vi "Reduce Files.vi"() -> ()   [LabVIEW 2015]
uses:
  <userlib>/_OpenG.lib/file/file.llb/Strip Path Extension - String__ogtk.vi
panel:
  out "spreadsheet string":string
  in  "Delete?":bool
  out "array 3":string[](array[string])
  out "array 2":string[](array[string])
  out "array":string[](array[string])
  # "UFileCrc32"
  # "INPUT: at blockdiagramm"
  # "Look out: some  *.pas files  do  not have a *.dcu file\nwhen included like\n{$I I_Connector_Diff.pas}"
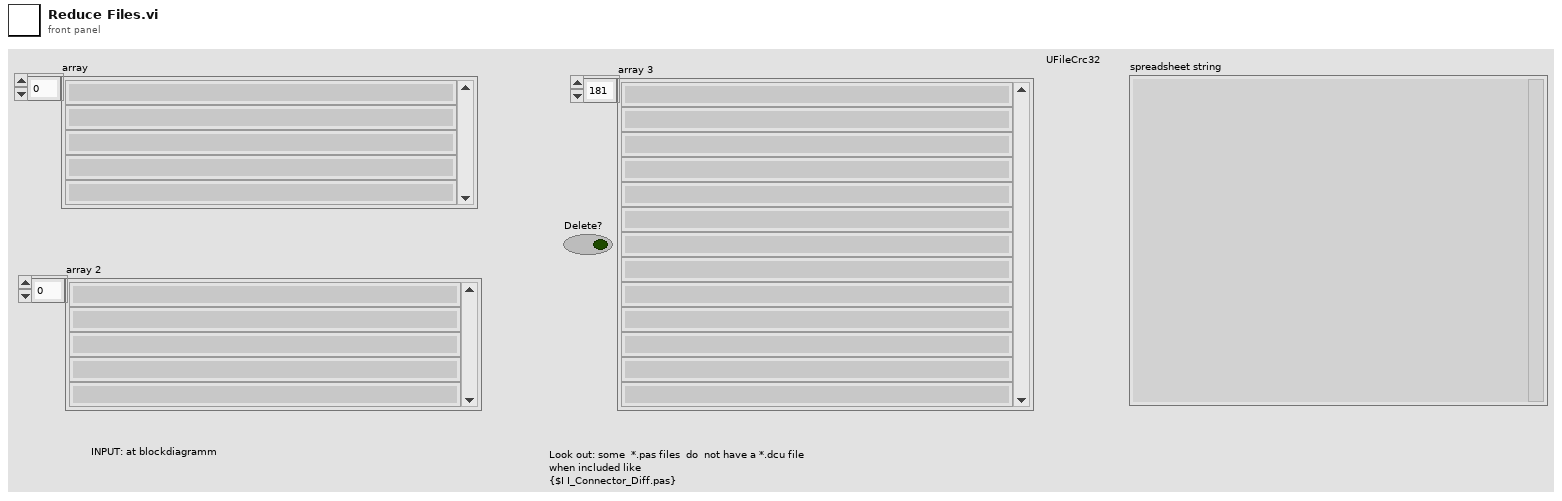
[diagram p1: front panel]
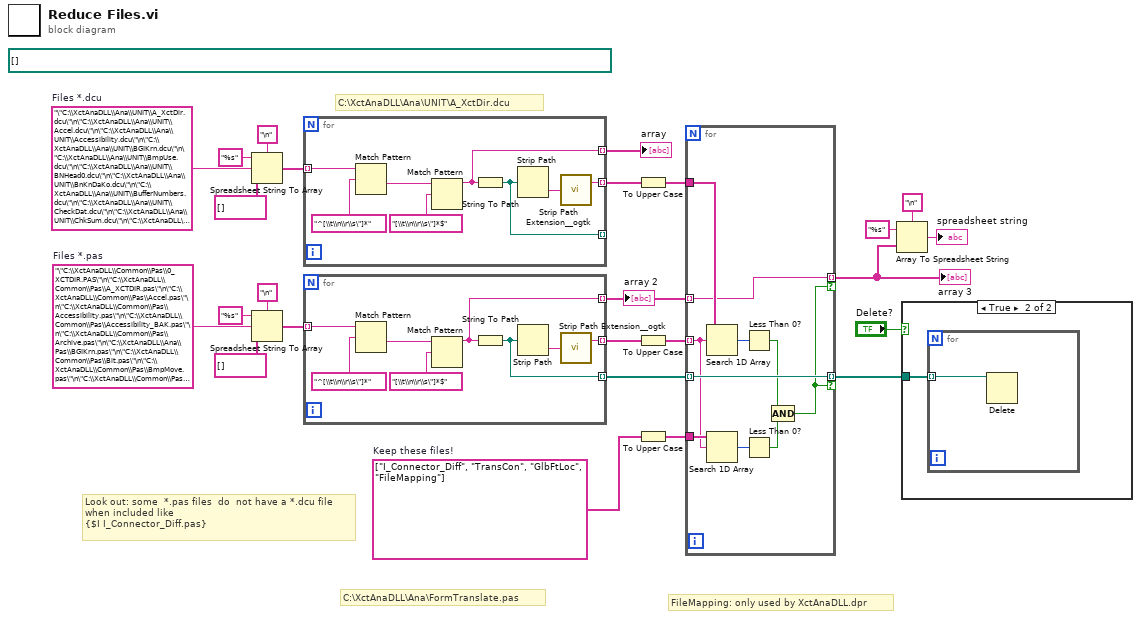
[diagram p0: block diagram]
diagram:
  w2 = string[] ["I_Connector_Diff", "TransCon", "GlbFtLoc", "FileMapping"]  # Keep these files!
  w19 = "\"C:\\XctAnaDLL\\Ana\\UNIT\\A_XctDir.dcu\"\n\"C:\\XctAnaDLL\\Ana\\UNIT\\Accel.dcu\"\n\"C:\\XctAnaDLL\\Ana\\UNIT\\Accessibility.dcu\"\n\"C:\\XctAnaDLL\\Ana\\UNIT\\BGIKrn.dcu\"\n\"C:\\XctAnaDLL\\Ana\\UNIT\\BmpUse.dcu\"\n\"C:\\XctAnaDLL\\Ana\\UNIT\\BNHead0.dcu\"\n\"C:\\XctAnaDLL\\Ana\\UNIT\\BnKnDaKo.dcu\"\n\"C:\\XctAnaDLL\\Ana\\UNIT\\BufferNumbers.dcu\"\n\"C:\\XctAnaDLL\\Ana\\UNIT\\CheckDat.dcu\"\n\"C:\\XctAnaDLL\\Ana\\UNIT\\ChkSum.dcu\"\n\"C:\\XctAnaDLL\\Ana\\UNIT\\ClientViewXctImagesUnit.dcu\"\n\"C:\\XctAnaDLL\\Ana\\UNIT\\ClipBrdUse.dcu\"\n\"C:\\XctAnaDLL\\Ana\\UNIT\\CodeFind.dcu\"\n\"C:\\XctAnaDLL\\Ana\\UNIT\\ColorDlgUse.dcu\"\n\"C:\\XctAnaDLL\\Ana\\UNIT\\ColorModels.dcu\"\n\"C:\\XctAnaDLL\\Ana\\UNIT\\ColorsPlus.dcu\"\n\"C:\\XctAnaDLL\\Ana\\UNIT\\ComNames.dcu\"\n\"C:\\XctAnaDLL\\Ana\\UNIT\\CRT.dcu\"\n\"C:\\XctAnaDLL\\Ana\\UNIT\\DebugForm.dcu\"\n\"C:\\XctAnaDLL\\Ana\\UNIT\\DefHTMLOpts.dcu\"\n\"C:\\XctAnaDLL\\Ana\\UNIT\\DelphiCrt.dcu\"\n\"C:\\XctAnaDLL\\Ana\\UNIT\\DialogsSecure.dcu\"\n\"C:\\XctAnaDLL\\Ana\\UNIT\\DIBTools.dcu\"\n\"C:\\XctAnaDLL\\Ana\\UNIT\\Dos.dcu\"\n\"C:\\XctAnaDLL\\Ana\\UNIT\\DosTimer.dcu\"\n\"C:\\XctAnaDLL\\Ana\\UNIT\\Draw.dcu\"\n\"C:\\XctAnaDLL\\Ana\\UNIT\\EE_Param.dcu\"\n\"C:\\XctAnaDLL\\Ana\\UNIT\\ErrConst.dcu\"\n\"C:\\XctAnaDLL\\Ana\\UNIT\\EventLogs.dcu\"\n\"C:\\XctAnaDLL\\Ana\\UNIT\\ExitTool.dcu\"\n\"C:\\XctAnaDLL\\Ana\\UNIT\\FemGlb.dcu\"\n\"C:\\XctAnaDLL\\Ana\\UNIT\\FemurPcForm1.dcu\"\n\"C:\\XctAnaDLL\\Ana\\UNIT\\FileUtils.dcu\"\n\"C:\\XctAnaDLL\\Ana\\UNIT\\FindEdge.dcu\"\n\"C:\\XctAnaDLL\\Ana\\UNIT\\FormatedList.dcu\"\n\"C:\\XctAnaDLL\\Ana\\UNIT\\FramePaint.dcu\"\n\"C:\\XctAnaDLL\\Ana\\UNIT\\frmBnLockPassWd.dcu\"\n\"C:\\XctAnaDLL\\Ana\\UNIT\\FrmXCTAbout.dcu\"\n\"C:\\XctAnaDLL\\Ana\\UNIT\\GlbDecs.dcu\"\n\"C:\\XctAnaDLL\\Ana\\UNIT\\GlbFT.dcu\"\n\"C:\\XctAnaDLL\\Ana\\UNIT\\GlbPath.dcu\"\n\"C:\\XctAnaDLL\\Ana\\UNIT\\GlbTools.dcu\"\n\"C:\\XctAnaDLL\\Ana\\UNIT\\GlbType.dcu\"\n\"C:\\XctAnaDLL\\Ana\\UNIT\\Graph0.dcu\"\n\"C:\\XctAnaDLL\\Ana\\UNIT\\GraphGlb.dcu\"\n\"C:\\XctAnaDLL\\Ana\\UNIT\\GraphicsExt.dcu\"\n\"C:\\XctAnaDLL\\Ana\\UNIT\\IOTools.dcu\"\n\"C:\\XctAnaDLL\\Ana\\UNIT\\JpgUse.dcu\"\n\"C:\\XctAnaDLL\\Ana\\UNIT\\KeyCodes.dcu\"\n\"C:\\XctAnaDLL\\Ana\\UNIT\\KeyState.dcu\"\n\"C:\\XctAnaDLL\\Ana\\UNIT\\Kn_Debug.dcu\"\n\"C:\\XctAnaDLL\\Ana\\UNIT\\KN_Err.dcu\"\n\"C:\\XctAnaDLL\\Ana\\UNIT\\KN_HLP.dcu\"\n\"C:\\XctAnaDLL\\Ana\\UNIT\\KN_Math.dcu\"\n\"C:\\XctAnaDLL\\Ana\\UNIT\\KN_MI.dcu\"\n\"C:\\XctAnaDLL\\Ana\\UNIT\\KN_NCONT.dcu\"\n\"C:\\XctAnaDLL\\Ana\\UNIT\\Kn_NGlb.dcu\"\n\"C:\\XctAnaDLL\\Ana\\UNIT\\KN_NSPLI.dcu\"\n\"C:\\XctAnaDLL\\Ana\\UNIT\\KN_PRINT.dcu\"\n\"C:\\XctAnaDLL\\Ana\\UNIT\\KN_ROI.dcu\"\n\"C:\\XctAnaDLL\\Ana\\UNIT\\KN_SetUp.dcu\"\n\"C:\\XctAnaDLL\\Ana\\UNIT\\KN_Slc.dcu\"\n\"C:\\XctAnaDLL\\Ana\\UNIT\\KN_TOPAZ.dcu\"\n\"C:\\XctAnaDLL\\Ana\\UNIT\\KnMulti.dcu\"\n\"C:\\XctAnaDLL\\Ana\\UNIT\\LabViewAna.dcu\"\n\"C:\\XctAnaDLL\\Ana\\UNIT\\LinTick0.dcu\"\n\"C:\\XctAnaDLL\\Ana\\UNIT\\LPCF_GLB.dcu\"\n\"C:\\XctAnaDLL\\Ana\\UNIT\\MemTools.dcu\"\n\"C:\\XctAnaDLL\\Ana\\UNIT\\MenuIds.dcu\"\n\"C:\\XctAnaDLL\\Ana\\UNIT\\MenuProc.dcu\"\n\"C:\\XctAnaDLL\\Ana\\UNIT\\MenuTool.dcu\"\n\"C:\\XctAnaDLL\\Ana\\UNIT\\MsgBox.dcu\"\n\"C:\\XctAnaDLL\\Ana\\UNIT\\Objects.dcu\"\n\"C:\\XctAnaDLL\\Ana\\UNIT\\Objects0.dcu\"\n\"C:\\XctAnaDLL\\Ana\\UNIT\\OrientDirUse.dcu\"\n\"C:\\XctAnaDLL\\Ana\\UNIT\\PCX.dcu\"\n\"C:\\XctAnaDLL\\Ana\\UNIT\\PntMath.dcu\"\n\"C:\\XctAnaDLL\\Ana\\UNIT\\PowerButton.dcu\"\n\"C:\\XctAnaDLL\\Ana\\UNIT\\PrinterGlb.dcu\"\n\"C:\\XctAnaDLL\\Ana\\UNIT\\PrintersFpu.dcu\"\n\"C:\\XctAnaDLL\\Ana\\UNIT\\PrintForm.dcu\"\n\"C:\\XctAnaDLL\\Ana\\UNIT\\ProgressBars.dcu\"\n\"C:\\XctAnaDLL\\Ana\\UNIT\\ReadPar.dcu\"\n\"C:\\XctAnaDLL\\Ana\\UNIT\\RectGlb.dcu\"\n\"C:\\XctAnaDLL\\Ana\\UNIT\\RoiDialog.dcu\"\n\"C:\\XctAnaDLL\\Ana\\UNIT\\RoiDialogTools.dcu\"\n\"C:\\XctAnaDLL\\Ana\\UNIT\\RoiMath.dcu\"\n\"C:\\XctAnaDLL\\Ana\\UNIT\\ScanIo0.dcu\"\n\"C:\\XctAnaDLL\\Ana\\UNIT\\SCRConst.dcu\"\n\"C:\\XctAnaDLL\\Ana\\UNIT\\SelectForm.dcu\"\n\"C:\\XctAnaDLL\\Ana\\UNIT\\SetDecimalPoint.dcu\"\n\"C:\\XctAnaDLL\\Ana\\UNIT\\SpinEdit2.dcu\"\n\"C:\\XctAnaDLL\\Ana\\UNIT\\StrTool.dcu\"\n\"C:\\XctAnaDLL\\Ana\\UNIT\\THaloEdi.dcu\"\n\"C:\\XctAnaDLL\\Ana\\UNIT\\THaloWin.dcu\"\n\"C:\\XctAnaDLL\\Ana\\UNIT\\ThreadView.dcu\"\n\"C:\\XctAnaDLL\\Ana\\UNIT\\TKeyApp.dcu\"\n\"C:\\XctAnaDLL\\Ana\\UNIT\\TMathobj.dcu\"\n\"C:\\XctAnaDLL\\Ana\\UNIT\\TMenuApp.dcu\"\n\"C:\\XctAnaDLL\\Ana\\UNIT\\TNHTOOL.dcu\"\n\"C:\\XctAnaDLL\\Ana\\UNIT\\Tools.dcu\"\n\"C:\\XctAnaDLL\\Ana\\UNIT\\Translate.dcu\"\n\"C:\\XctAnaDLL\\Ana\\UNIT\\TransX.dcu\"\n\"C:\\XctAnaDLL\\Ana\\UNIT\\TurbExt1.dcu\"\n\"C:\\XctAnaDLL\\Ana\\UNIT\\TurboToDelphi.dcu\"\n\"C:\\XctAnaDLL\\Ana\\UNIT\\TypesUse.dcu\"\n\"C:\\XctAnaDLL\\Ana\\UNIT\\UBnLockWin.dcu\"\n\"C:\\XctAnaDLL\\Ana\\UNIT\\UFileCrc32.dcu\"\n\"C:\\XctAnaDLL\\Ana\\UNIT\\UfrmRefReport.dcu\"\n\"C:\\XctAnaDLL\\Ana\\UNIT\\UfrmShowRef.dcu\"\n\"C:\\XctAnaDLL\\Ana\\UNIT\\UMsgDelay.dcu\"\n\"C:\\XctAnaDLL\\Ana\\UNIT\\UniDIB.dcu\"\n\"C:\\XctAnaDLL\\Ana\\UNIT\\UReadSet.dcu\"\n\"C:\\XctAnaDLL\\Ana\\UNIT\\UseDelphi.dcu\"\n\"C:\\XctAnaDLL\\Ana\\UNIT\\UTA_CBD.dcu\"\n\"C:\\XctAnaDLL\\Ana\\UNIT\\UtAna.dcu\"\n\"C:\\XctAnaDLL\\Ana\\UNIT\\UTAna1.dcu\"\n\"C:\\XctAnaDLL\\Ana\\UNIT\\UTAROI.dcu\"\n\"C:\\XctAnaDLL\\Ana\\UNIT\\UTArray.dcu\"\n\"C:\\XctAnaDLL\\Ana\\UNIT\\UTBuffer.dcu\"\n\"C:\\XctAnaDLL\\Ana\\UNIT\\UTColDlg.dcu\"\n\"C:\\XctAnaDLL\\Ana\\UNIT\\UTColor.dcu\"\n\"C:\\XctAnaDLL\\Ana\\UNIT\\UTDBI.dcu\"\n\"C:\\XctAnaDLL\\Ana\\UNIT\\UtFilt0.dcu\"\n\"C:\\XctAnaDLL\\Ana\\UNIT\\UtFilter.dcu\"\n\"C:\\XctAnaDLL\\Ana\\UNIT\\UTGenOb.dcu\"\n\"C:\\XctAnaDLL\\Ana\\UNIT\\UTGENROI.dcu\"\n\"C:\\XctAnaDLL\\Ana\\UNIT\\UTGrpRes.dcu\"\n\"C:\\XctAnaDLL\\Ana\\UNIT\\UtIni.dcu\"\n\"C:\\XctAnaDLL\\Ana\\UNIT\\UTIP.dcu\"\n\"C:\\XctAnaDLL\\Ana\\UNIT\\UTKnApp.dcu\"\n\"C:\\XctAnaDLL\\Ana\\UNIT\\UTKnApp0.dcu\"\n\"C:\\XctAnaDLL\\Ana\\UNIT\\UTKNAPP1.dcu\"\n\"C:\\XctAnaDLL\\Ana\\UNIT\\UTKNAPP2.dcu\"\n\"C:\\XctAnaDLL\\Ana\\UNIT\\UtKnPane.dcu\"\n\"C:\\XctAnaDLL\\Ana\\UNIT\\UTParam.dcu\"\n\"C:\\XctAnaDLL\\Ana\\UNIT\\UTRef.dcu\"\n\"C:\\XctAnaDLL\\Ana\\UNIT\\UTRes.dcu\"\n\"C:\\XctAnaDLL\\Ana\\UNIT\\UTStd.dcu\"\n\"C:\\XctAnaDLL\\Ana\\UNIT\\VidLine.dcu\"\n\"C:\\XctAnaDLL\\Ana\\UNIT\\ViewQLim.dcu\"\n\"C:\\XctAnaDLL\\Ana\\UNIT\\ViewScreens.dcu\"\n\"C:\\XctAnaDLL\\Ana\\UNIT\\ViewXctImages.dcu\"\n\"C:\\XctAnaDLL\\Ana\\UNIT\\ViewXctServerClientGlb.dcu\"\n\"C:\\XctAnaDLL\\Ana\\UNIT\\WindowsEx.dcu\"\n\"C:\\XctAnaDLL\\Ana\\UNIT\\WinTmr.dcu\"\n\"C:\\XctAnaDLL\\Ana\\UNIT\\WinTools.dcu\"\n\"C:\\XctAnaDLL\\Ana\\UNIT\\WM_AddMessages.dcu\"\n\"C:\\XctAnaDLL\\Ana\\UNIT\\XctVersion.dcu\"\n\"C:\\XctAnaDLL\\Ana\\UNIT\\XGlb.dcu\"\n\"C:\\XctAnaDLL\\Ana\\UNIT\\XMeasGrp.dcu\""  # Files *.dcu
  w18 = "\"C:\\XctAnaDLL\\Common\\Pas\\0_XCTDIR.PAS\"\n\"C:\\XctAnaDLL\\Common\\Pas\\A_XCTDIR.pas\"\n\"C:\\XctAnaDLL\\Common\\Pas\\Accel.pas\"\n\"C:\\XctAnaDLL\\Common\\Pas\\Accessibility.pas\"\n\"C:\\XctAnaDLL\\Common\\Pas\\Accessibility_BAK.pas\"\n\"C:\\XctAnaDLL\\Common\\Pas\\Archive.pas\"\n\"C:\\XctAnaDLL\\Ana\\Pas\\BGIKrn.pas\"\n\"C:\\XctAnaDLL\\Common\\Pas\\Bit.pas\"\n\"C:\\XctAnaDLL\\Common\\Pas\\BmpMove.pas\"\n\"C:\\XctAnaDLL\\Common\\Pas\\BmpStack.pas\"\n\"C:\\XctAnaDLL\\Common\\Pas\\BmpUse.pas\"\n\"C:\\XctAnaDLL\\Common\\Pas\\BNHead0.pas\"\n\"C:\\XctAnaDLL\\Ana\\Pas\\BNKEY0.pas\"\n\"C:\\XctAnaDLL\\Ana\\Pas\\BnKnDaKo.pas\"\n\"C:\\XctAnaDLL\\Ana\\Pas\\BNLOCK.pas\"\n\"C:\\XctAnaDLL\\Ana\\Pas\\BufferNumbers.pas\"\n\"C:\\XctAnaDLL\\Ana\\Pas\\BufferNumbers_2.pas\"\n\"C:\\XctAnaDLL\\Ana\\Pas\\Calc.pas\"\n\"C:\\XctAnaDLL\\Common\\Pas\\CheckDat.pas\"\n\"C:\\XctAnaDLL\\Common\\Pas\\CheckPrevious.pas\"\n\"C:\\XctAnaDLL\\Ana\\Pas\\CHK540UP.PAS\"\n\"C:\\XctAnaDLL\\Common\\Pas\\ChkSum.pas\"\n\"C:\\XctAnaDLL\\Ana\\Pas\\ChngSide.pas\"\n\"C:\\XctAnaDLL\\Common\\Pas\\ClientViewXctImagesUnit.pas\"\n\"C:\\XctAnaDLL\\Common\\Pas\\ClipBrdUse.pas\"\n\"C:\\XctAnaDLL\\Ana\\Pas\\cmConst.pas\"\n\"C:\\XctAnaDLL\\Ana\\Pas\\CMDPARAM.PAS\"\n\"C:\\XctAnaDLL\\Common\\Pas\\CodeFind.pas\"\n\"C:\\XctAnaDLL\\Common\\Pas\\ColorDlgUse.pas\"\n\"C:\\XctAnaDLL\\Common\\Pas\\ColorModels.pas\"\n\"C:\\XctAnaDLL\\Common\\Pas\\ColorsPlus.pas\"\n\"C:\\XctAnaDLL\\Info\\TempTest\\COMAC000_Msk.pas\"\n\"C:\\XctAnaDLL\\Info\\TempTest\\COMACFEM_Msk.pas\"\n\"C:\\XctAnaDLL\\Common\\Pas\\ComNames.pas\"\n\"C:\\XctAnaDLL\\Common\\Pas\\ComparePathes.pas\"\n\"C:\\XctAnaDLL\\Common\\Pas\\Complexs.pas\"\n\"C:\\XctAnaDLL\\Ana\\Pas\\CONF.PAS\"\n\"C:\\XctAnaDLL\\Common\\Pas\\ControlsUse.pas\"\n\"C:\\XctAnaDLL\\Common\\Pas\\Crt.pas\"\n\"C:\\XctAnaDLL\\Ana\\Pas\\CSV2PAL.pas\"\n\"C:\\XctAnaDLL\\Ana\\Pas\\csvread.pas\"\n\"C:\\XctAnaDLL\\Ana\\Pas\\CSVSTAT.pas\"\n\"C:\\XctAnaDLL\\Ana\\Pas\\CVDOSTXT.PAS\"\n\"C:\\XctAnaDLL\\Common\\Pas\\DataBaseXct.pas\"\n\"C:\\XctAnaDLL\\Common\\Pas\\DebInit.pas\"\n\"C:\\XctAnaDLL\\Common\\Pas\\DebugForm.pas\"\n\"C:\\XctAnaDLL\\Ana\\Pas\\DefDrvs.pas\"\n\"C:\\XctAnaDLL\\Common\\Pas\\DefHTMLOpts.pas\"\n\"C:\\XctAnaDLL\\Common\\Pas\\DelphiCrt.pas\"\n\"C:\\XctAnaDLL\\Common\\Pas\\DialogsSecure.pas\"\n\"C:\\XctAnaDLL\\Common\\Pas\\DIBTools.pas\"\n\"C:\\XctAnaDLL\\Common\\Pas\\DirTool.pas\"\n\"C:\\XctAnaDLL\\Common\\Pas\\DiskTyp.pas\"\n\"C:\\XctAnaDLL\\Common\\Pas\\DlgDeltaTime.pas\"\n\"C:\\XctAnaDLL\\Ana\\Pas\\Do540up.pas\"\n\"C:\\XctAnaDLL\\Ana\\Pas\\DoModify.pas\"\n\"C:\\XctAnaDLL\\Common\\Pas\\Dos.pas\"\n\"C:\\XctAnaDLL\\Common\\Pas\\DosGlb.pas\"\n\"C:\\XctAnaDLL\\Common\\Pas\\DosTimer.pas\"\n\"C:\\XctAnaDLL\\Common\\Pas\\Draw.pas\"\n\"C:\\XctAnaDLL\\Common\\Pas\\DrawGridDialog.pas\"\n\"C:\\XctAnaDLL\\Ana\\Pas\\DUMMY.PAS\"\n\"C:\\XctAnaDLL\\Common\\Pas\\EE_Param.pas\"\n\"C:\\XctAnaDLL\\Common\\Pas\\EE_Param_RW.pas\"\n\"C:\\XctAnaDLL\\Common\\Pas\\EE_Param_Tools.pas\"\n\"C:\\XctAnaDLL\\Common\\Pas\\ErrConst.pas\"\n\"C:\\XctAnaDLL\\Common\\Pas\\EventLog.pas\"\n\"C:\\XctAnaDLL\\Common\\Pas\\EventLogs.pas\"\n\"C:\\XctAnaDLL\\Ana\\Pas\\ExGraph.pas\"\n\"C:\\XctAnaDLL\\Common\\Pas\\ExitTool.pas\"\n\"C:\\XctAnaDLL\\Ana\\Pas\\EXTPLUS.pas\"\n\"C:\\XctAnaDLL\\Ana\\Pas\\FCOUNT.pas\"\n\"C:\\XctAnaDLL\\Common\\Pas\\FemGlb.pas\"\n\"C:\\XctAnaDLL\\Common\\Pas\\FemurPcForm1.pas\"\n\"C:\\XctAnaDLL\\Common\\Pas\\FFTs.pas\"\n\"C:\\XctAnaDLL\\Delphi\\FileMapping.pas\"\n\"C:\\XctAnaDLL\\Common\\Pas\\FileUtils.pas\"\n\"C:\\XctAnaDLL\\Ana\\Pas\\FindEdge.pas\"\n\"C:\\XctAnaDLL\\Common\\Pas\\FirFilter.pas\"\n\"C:\\XctAnaDLL\\Common\\Pas\\FormatedList.pas\"\n\"C:\\XctAnaDLL\\Common\\Pas\\FormatTools.pas\"\n\"C:\\XctAnaDLL\\Ana\\Pas\\formLoopEdit.pas\"\n\"C:\\XctAnaDLL\\Common\\Pas\\FormMountImage.pas\"\n\"C:\\XctAnaDLL\\Ana\\FormTranslate.pas\"\n\"C:\\XctAnaDLL\\Common\\Pas\\Fourier.pas\"\n\"C:\\XctAnaDLL\\Common\\Pas\\FramePaint.pas\"\n\"C:\\XctAnaDLL\\Common\\Pas\\Frames.pas\"\n\"C:\\XctAnaDLL\\Common\\Pas\\FrameScrolledImage.pas\"\n\"C:\\XctAnaDLL\\Common\\Pas\\FrameScrolledImageTool.pas\"\n\"C:\\XctAnaDLL\\Common\\Pas\\FrameToolRect.pas\"\n\"C:\\XctAnaDLL\\Common\\Pas\\frmBnLockPassWd.pas\"\n\"C:\\XctAnaDLL\\Common\\Pas\\frmHexEdit_U.pas\"\n\"C:\\XctAnaDLL\\Common\\Pas\\frmImage.pas\"\n\"C:\\XctAnaDLL\\Common\\Pas\\frmOptsFilesHyperlink.pas\"\n\"C:\\XctAnaDLL\\Common\\Pas\\FrmXCTAbout.pas\"\n\"C:\\XctAnaDLL\\Common\\Pas\\GdiPlusUse.pas\"\n\"C:\\XctAnaDLL\\Common\\Pas\\GeoTools.pas\"\n\"C:\\XctAnaDLL\\Common\\Pas\\GetMovit.pas\"\n\"C:\\XctAnaDLL\\Common\\Pas\\GetTast.pas\"\n\"C:\\XctAnaDLL\\Common\\Pas\\GIFImage.pas\"\n\"C:\\XctAnaDLL\\Common\\Pas\\Glb.pas\"\n\"C:\\XctAnaDLL\\Common\\Pas\\GlbDecs.pas\"\n\"C:\\XctAnaDLL\\Common\\Pas\\GlbFT.pas\"\n\"C:\\XctAnaDLL\\Ana\\Pas\\GlbFtLoc.Pas\"\n\"C:\\XctAnaDLL\\Common\\Pas\\GlbFtLoc.Pas\"\n\"C:\\XctAnaDLL\\Common\\Pas\\GlbHotKey.pas\"\n\"C:\\XctAnaDLL\\Common\\Pas\\GlbKey.pas\"\n\"C:\\XctAnaDLL\\Common\\Pas\\GlbPath.pas\"\n\"C:\\XctAnaDLL\\Common\\Pas\\Glbtools.pas\"\n\"C:\\XctAnaDLL\\Common\\Pas\\GlbType.pas\"\n\"C:\\XctAnaDLL\\Ana\\Pas\\GoXctDir.pas\"\n\"C:\\XctAnaDLL\\Common\\Pas\\Gr_Crt.pas\"\n\"C:\\XctAnaDLL\\Common\\Pas\\Graph0.pas\"\n\"C:\\XctAnaDLL\\Common\\Pas\\GraphGlb.pas\"\n\"C:\\XctAnaDLL\\Common\\Pas\\GraphicsExt.pas\"\n\"C:\\XctAnaDLL\\Common\\Pas\\GridBasic.pas\"\n\"C:\\XctAnaDLL\\Ana\\Pas\\HelpFile.pas\"\n\"C:\\XctAnaDLL\\Common\\Pas\\I_Connector_Diff.pas\"\n\"C:\\XctAnaDLL\\Common\\Pas\\IfTool.pas\"\n\"C:\\XctAnaDLL\\Common\\Pas\\ImgBuf.pas\"\n\"C:\\XctAnaDLL\\Common\\Pas\\ImgMeasTools.pas\"\n\"C:\\XctAnaDLL\\Common\\Pas\\ImgOverview.pas\"\n\"C:\\XctAnaDLL\\Common\\Pas\\IniFilesUse.pas\"\n\"C:\\XctAnaDLL\\Common\\Pas\\IntChar.pas\"\n\"C:\\XctAnaDLL\\Ana\\Pas\\Intopaz.pas\"\n\"C:\\XctAnaDLL\\Common\\Pas\\IoErr.pas\"\n\"C:\\XctAnaDLL\\Common\\Pas\\IOTools.pas\"\n\"C:\\XctAnaDLL\\Common\\Pas\\JobParameter.pas\"\n\"C:\\XctAnaDLL\\JPEG\\jpeg.pas\"\n\"C:\\XctAnaDLL\\Common\\Pas\\JpgUse.pas\"\n\"C:\\XctAnaDLL\\Common\\Pas\\KeyCodes.pas\"\n\"C:\\XctAnaDLL\\Ana\\Pas\\Keys.pas\"\n\"C:\\XctAnaDLL\\Common\\Pas\\KeyState.pas\"\n\"C:\\XctAnaDLL\\Ana\\Pas\\Kn_Debug.pas\"\n\"C:\\XctAnaDLL\\Ana\\Pas\\KN_Err.pas\"\n\"C:\\XctAnaDLL\\Ana\\Pas\\KN_HLP.pas\"\n\"C:\\XctAnaDLL\\Ana\\Pas\\KN_Intpz.pas\"\n\"C:\\XctAnaDLL\\Ana\\Pas\\Kn_Math.pas\"\n\"C:\\XctAnaDLL\\Ana\\Pas\\KN_MI.pas\"\n\"C:\\XctAnaDLL\\Ana\\Pas\\KN_NCONT.pas\"\n\"C:\\XctAnaDLL\\Ana\\Pas\\Kn_NGlb.pas\"\n\"C:\\XctAnaDLL\\Ana\\Pas\\KN_NSPLI.pas\"\n\"C:\\XctAnaDLL\\Ana\\Pas\\KN_PRINT.pas\"\n\"C:\\XctAnaDLL\\Ana\\Pas\\KN_ROI.pas\"\n\"C:\\XctAnaDLL\\Ana\\Pas\\KN_SetUp.pas\"\n\"C:\\XctAnaDLL\\Ana\\Pas\\Kn_Slc.pas\"\n\"C:\\XctAnaDLL\\Ana\\Pas\\KN_SLC0.pas\"\n\"C:\\XctAnaDLL\\Ana\\Pas\\KN_TOPAZ.pas\"\n\"C:\\XctAnaDLL\\Ana\\Pas\\KNHLP.pas\"\n\"C:\\XctAnaDLL\\Ana\\Pas\\KnMulti.PAS\"\n\"C:\\XctAnaDLL\\Ana\\Pas\\LabViewAna.pas\"\n\"C:\\XctAnaDLL\\Common\\Pas\\License.pas\"\n\"C:\\XctAnaDLL\\Ana\\Pas\\LicensNo.pas\"\n\"C:\\XctAnaDLL\\Ana\\Pas\\LinTick0.pas\"\n\"C:\\XctAnaDLL\\Ana\\Pas\\loopcfg.pas\"\n\"C:\\XctAnaDLL\\Ana\\Pas\\LoopEditIo.pas\"\n\"C:\\XctAnaDLL\\Ana\\Pas\\LPCF_GLB.pas\"\n\"C:\\XctAnaDLL\\Ana\\Pas\\Lpcftool.pas\"\n\"C:\\XctAnaDLL\\Common\\Pas\\Lv_Tools.pas\"\n\"C:\\XctAnaDLL\\Common\\Pas\\Mail.pas\"\n\"C:\\XctAnaDLL\\Common\\Pas\\MathTool.pas\"\n\"C:\\XctAnaDLL\\Common\\Pas\\MathUse.pas\"\n\"C:\\XctAnaDLL\\Ana\\Pas\\MemTools.pas\"\n\"C:\\XctAnaDLL\\Ana\\Pas\\MenuCons.pas\"\n\"C:\\XctAnaDLL\\Common\\Pas\\MenuIds.pas\"\n\"C:\\XctAnaDLL\\Ana\\Pas\\MenuProc.pas\"\n\"C:\\XctAnaDLL\\Ana\\Pas\\MenuTool.pas\"\n\"C:\\XctAnaDLL\\Common\\Pas\\Minimize.pas\"\n\"C:\\XctAnaDLL\\Common\\Pas\\MsgBox.pas\"\n\"C:\\XctAnaDLL\\Ana\\Pas\\MYREN.pas\"\n\"C:\\XctAnaDLL\\Ana\\Pas\\MyValid.pas\"\n\"C:\\XctAnaDLL\\Ana\\Pas\\NETDEBUG.PAS\"\n\"C:\\XctAnaDLL\\Common\\Pas\\NoXctDir.pas\"\n\"C:\\XctAnaDLL\\Common\\Pas\\Objects.pas\"\n\"C:\\XctAnaDLL\\Common\\Pas\\Objects0.pas\"\n\"C:\\XctAnaDLL\\Common\\Pas\\ObjectsP.pas\"\n\"C:\\XctAnaDLL\\Ana\\Pas\\OEMANSI.PAS\"\n\"C:\\XctAnaDLL\\Ana\\Pas\\OLDVER.pas\"\n\"C:\\XctAnaDLL\\Common\\Pas\\OrientDirUse.pas\"\n\"C:\\XctAnaDLL\\Ana\\Pas\\OVERTYP.pas\"\n\"C:\\XctAnaDLL\\Ana\\Pas\\PAL2CSV.pas\"\n\"C:\\XctAnaDLL\\Common\\Pas\\PauseMsg.pas\"\n\"C:\\XctAnaDLL\\Common\\Pas\\PCX.pas\"\n\"C:\\XctAnaDLL\\Ana\\Pas\\Phan_DLG.pas\"\n\"C:\\XctAnaDLL\\Ana\\Pas\\PifTools.pas\"\n\"C:\\XctAnaDLL\\Common\\Pas\\PntMath.pas\"\n\"C:\\XctAnaDLL\\Common\\Pas\\PowerButton.pas\"\n\"C:\\XctAnaDLL\\Common\\Pas\\PowerButton2.pas\"\n\"C:\\XctAnaDLL\\Common\\Pas\\PrinterGlb.pas\"\n\"C:\\XctAnaDLL\\Common\\Pas\\PrintersFpu.pas\"\n\"C:\\XctAnaDLL\\Common\\Pas\\PrintForm.pas\"\n\"C:\\XctAnaDLL\\Common\\Pas\\PrintFormatted.pas\"\n\"C:\\XctAnaDLL\\Common\\Pas\\PrintTable.pas\"\n\"C:\\XctAnaDLL\\Common\\Pas\\PrnFormatedPages.pas\"\n\"C:\\XctAnaDLL\\Common\\Pas\\ProgressBars.pas\"\n\"C:\\XctAnaDLL\\Common\\Pas\\ReadPar.pas\"\n\"C:\\XctAnaDLL\\Common\\Pas\\Rectangles.pas\"\n\"C:\\XctAnaDLL\\Common\\Pas\\RectGlb.pas\"\n\"C:\\XctAnaDLL\\Ana\\Pas\\Resloop.pas\"\n\"C:\\XctAnaDLL\\Common\\Pas\\ResUse.pas\"\n\"C:\\XctAnaDLL\\Ana\\Pas\\rfdbio.pas\"\n\"C:\\XctAnaDLL\\Common\\Pas\\RichEditUse.pas\"\n\"C:\\XctAnaDLL\\Ana\\Pas\\RoiDialog.pas\"\n\"C:\\XctAnaDLL\\Ana\\Pas\\RoiDialogTools.pas\"\n\"C:\\XctAnaDLL\\Ana\\Pas\\RoiMath.pas\"\n\"C:\\XctAnaDLL\\Common\\Pas\\RollImage.pas\"\n\"C:\\XctAnaDLL\\Common\\Pas\\Round1.pas\"\n\"C:\\XctAnaDLL\\Common\\Pas\\SaverDelphi.pas\"\n\"C:\\XctAnaDLL\\Common\\Pas\\ScanIo0.pas\"\n\"C:\\XctAnaDLL\\Ana\\Pas\\ScrConst.pas\"\n\"C:\\XctAnaDLL\\Ana\\Pas\\Search.pas\"\n\"C:\\XctAnaDLL\\Common\\Pas\\SelectForm.pas\"\n\"C:\\XctAnaDLL\\Common\\Pas\\SerialPortThread.pas\"\n\"C:\\XctAnaDLL\\Common\\Pas\\SerialPortXct.pas\"\n\"C:\\XctAnaDLL\\Common\\Pas\\ServerViewXctImagesUnit.pas\"\n\"C:\\XctAnaDLL\\Ana\\Pas\\SetAvDrv.pas\"\n\"C:\\XctAnaDLL\\Common\\Pas\\SetDecimalPoint.pas\"\n\"C:\\XctAnaDLL\\Ana\\Pas\\SETINI.pas\"\n\"C:\\XctAnaDLL\\Common\\Pas\\ShellLink.pas\"\n\"C:\\XctAnaDLL\\Ana\\Pas\\sparcnst.pas\"\n\"C:\\XctAnaDLL\\Common\\Pas\\SpinEditFloat.pas\"\n\"C:\\XctAnaDLL\\Common\\Pas\\Splines.pas\"\n\"C:\\XctAnaDLL\\Common\\Pas\\StartMeasDialogs.pas\"\n\"C:\\XctAnaDLL\\Common\\Pas\\StreamUse.pas\"\n\"C:\\XctAnaDLL\\Common\\Pas\\StrTool.pas\"\n\"C:\\XctAnaDLL\\Common\\Pas\\SysUse.pas\"\n\"C:\\XctAnaDLL\\Ana\\Pas\\T.PAS\"\n\"C:\\XctAnaDLL\\Ana\\Pas\\T2.PAS\"\n\"C:\\XctAnaDLL\\Ana\\Pas\\T3.PAS\"\n\"C:\\XctAnaDLL\\Ana\\Pas\\T22.PAS\"\n\"C:\\XctAnaDLL\\Ana\\Pas\\TAPP.PAS\"\n\"C:\\XctAnaDLL\\Ana\\Pas\\TAPP2.PAS\"\n\"C:\\XctAnaDLL\\Ana\\Pas\\TDrives.pas\"\n\"C:\\XctAnaDLL\\Common\\Pas\\TeeUse.pas\"\n\"C:\\XctAnaDLL\\Ana\\Pas\\TF.PAS\"\n\"C:\\XctAnaDLL\\Ana\\Pas\\THaloEdi.pas\"\n\"C:\\XctAnaDLL\\Ana\\Pas\\THaloWin.pas\"\n\"C:\\XctAnaDLL\\Common\\Pas\\ThreadView.pas\"\n\"C:\\XctAnaDLL\\Common\\Pas\\TKeyApp.pas\"\n\"C:\\XctAnaDLL\\Ana\\Pas\\TLIST.PAS\"\n\"C:\\XctAnaDLL\\Ana\\Pas\\TMathobj.pas\"\n\"C:\\XctAnaDLL\\Ana\\Pas\\TMenuApp.pas\"\n\"C:\\XctAnaDLL\\Ana\\Pas\\TNHTool.pas\"\n\"C:\\XctAnaDLL\\Common\\Pas\\Tools.pas\"\n\"C:\\XctAnaDLL\\Ana\\Pas\\TRANSCON.PAS\"\n\"C:\\XctAnaDLL\\Common\\Pas\\TRANSCON.PAS\"\n\"C:\\XctAnaDLL\\Common\\Pas\\Translate.pas\"\n\"C:\\XctAnaDLL\\Ana\\TranslateData.pas\"\n\"C:\\XctAnaDLL\\Common\\Pas\\TransX.pas\"\n\"C:\\XctAnaDLL\\Common\\Pas\\TstShlObj.pas\"\n\"C:\\XctAnaDLL\\Ana\\Pas\\TT.PAS\"\n\"C:\\XctAnaDLL\\Ana\\Pas\\TTGRAPHS.PAS\"\n\"C:\\XctAnaDLL\\Ana\\Pas\\TTT.PAS\"\n\"C:\\XctAnaDLL\\Common\\Pas\\TurbExt1.pas\"\n\"C:\\XctAnaDLL\\Common\\Pas\\TurboToDelphi.pas\"\n\"C:\\XctAnaDLL\\Ana\\Pas\\tvedit.pas\"\n\"C:\\XctAnaDLL\\Common\\Pas\\Type_s.pas\"\n\"C:\\XctAnaDLL\\Common\\Pas\\TypesUse.pas\"\n\"C:\\XctAnaDLL\\Common\\Pas\\TZBOXES.pas\"\n\"C:\\XctAnaDLL\\Ana\\Pas\\UBNLock.pas\"\n\"C:\\XctAnaDLL\\Common\\Pas\\UBnlockWin.pas\"\n\"C:\\XctAnaDLL\\Common\\Pas\\UFileCRC32.pas\"\n\"C:\\XctAnaDLL\\Common\\Pas\\UfrmClipBoardTools.pas\"\n\"C:\\XctAnaDLL\\Common\\Pas\\UfrmErrBox.pas\"\n\"C:\\XctAnaDLL\\Ana\\Pas\\UfrmRefReport.pas\"\n\"C:\\XctAnaDLL\\Ana\\Pas\\UfrmShowRef.pas\"\n\"C:\\XctAnaDLL\\Ana\\Pas\\UGetKey.pas\"\n\"C:\\XctAnaDLL\\Common\\Pas\\UMsgDelay.pas\"\n\"C:\\XctAnaDLL\\Common\\Pas\\UniDIB.pas\"\n\"C:\\XctAnaDLL\\Info\\TempTest\\Unit1.pas\"\n\"C:\\XctAnaDLL\\Ana\\Pas\\UParUpd.pas\"\n\"C:\\XctAnaDLL\\Ana\\Pas\\UPD51X.pas\"\n\"C:\\XctAnaDLL\\Ana\\Pas\\UPD52X.pas\"\n\"C:\\XctAnaDLL\\Ana\\Pas\\UReadSet.pas\"\n\"C:\\XctAnaDLL\\Common\\Pas\\UseDelphi.pas\"\n\"C:\\XctAnaDLL\\Common\\Pas\\UseDragDrop.pas\"\n\"C:\\XctAnaDLL\\Common\\Pas\\UseGlbHotKeys.pas\"\n\"C:\\XctAnaDLL\\Common\\Pas\\UseList.pas\"\n\"C:\\XctAnaDLL\\Ana\\Pas\\UseUTIP_2.pas\"\n\"C:\\XctAnaDLL\\Ana\\Pas\\UTA_CBD.pas\"\n\"C:\\XctAnaDLL\\Ana\\Pas\\UTANA.pas\"\n\"C:\\XctAnaDLL\\Ana\\Pas\\UTAna1.pas\"\n\"C:\\XctAnaDLL\\Ana\\Pas\\UTAROI.pas\"\n\"C:\\XctAnaDLL\\Ana\\Pas\\UTArray.pas\"\n\"C:\\XctAnaDLL\\Ana\\Pas\\UTBuffer.pas\"\n\"C:\\XctAnaDLL\\Ana\\Pas\\UTBuffer_2.pas\"\n\"C:\\XctAnaDLL\\Ana\\Pas\\UTCOLDLG.pas\"\n\"C:\\XctAnaDLL\\Ana\\Pas\\UTColor.pas\"\n\"C:\\XctAnaDLL\\Ana\\Pas\\UTDBI.pas\"\n\"C:\\XctAnaDLL\\Common\\Pas\\UtFilt0.pas\"\n\"C:\\XctAnaDLL\\Ana\\Pas\\UTFilter.pas\"\n\"C:\\XctAnaDLL\\Common\\Pas\\UTGenOb.pas\"\n\"C:\\XctAnaDLL\\Ana\\Pas\\UTGENROI.pas\"\n\"C:\\XctAnaDLL\\Ana\\Pas\\UTGrpRes.pas\"\n\"C:\\XctAnaDLL\\Common\\Pas\\UtIni.pas\"\n\"C:\\XctAnaDLL\\Ana\\UTINI_Console.pas\"\n\"C:\\XctAnaDLL\\Ana\\Pas\\UTIP.pas\"\n\"C:\\XctAnaDLL\\Ana\\Pas\\UTIP_2.pas\"\n\"C:\\XctAnaDLL\\Ana\\Pas\\UTKnApp.pas\"\n\"C:\\XctAnaDLL\\Ana\\Pas\\UTKNApp0.pas\"\n\"C:\\XctAnaDLL\\Ana\\Pas\\UTKNAPP1.pas\"\n\"C:\\XctAnaDLL\\Ana\\Pas\\UTKNAPP2.pas\"\n\"C:\\XctAnaDLL\\Ana\\Pas\\UtKnPane.pas\"\n\"C:\\XctAnaDLL\\Ana\\Pas\\UTParam.pas\"\n\"C:\\XctAnaDLL\\Ana\\Pas\\UTRef.pas\"\n\"C:\\XctAnaDLL\\Ana\\Pas\\UTRes.pas\"\n\"C:\\XctAnaDLL\\Ana\\Pas\\UTStd.pas\"\n\"C:\\XctAnaDLL\\Ana\\Pas\\UTTABEL.PAS\"\n\"C:\\XctAnaDLL\\Common\\Pas\\UViewErrScr.pas\"\n\"C:\\XctAnaDLL\\Common\\Pas\\VideHook.pas\"\n\"C:\\XctAnaDLL\\Ana\\Pas\\VidLine.pas\"\n\"C:\\XctAnaDLL\\Common\\Pas\\VidLine01.pas\"\n\"C:\\XctAnaDLL\\Common\\Pas\\ViewGrid.pas\"\n\"C:\\XctAnaDLL\\Common\\Pas\\ViewGridUse.pas\"\n\"C:\\XctAnaDLL\\Ana\\Pas\\ViewQLim.pas\"\n\"C:\\XctAnaDLL\\Common\\Pas\\ViewScreens.pas\"\n\"C:\\XctAnaDLL\\Common\\Pas\\ViewXctImages.pas\"\n\"C:\\XctAnaDLL\\Common\\Pas\\ViewXctServerClientGlb.pas\"\n\"C:\\XctAnaDLL\\Info\\TempTest\\WDBIMSK.PAS\"\n\"C:\\XctAnaDLL\\Common\\Pas\\WindowsEx.pas\"\n\"C:\\XctAnaDLL\\Common\\WinFolders.pas\"\n\"C:\\XctAnaDLL\\Common\\Pas\\WinMessagDialog.pas\"\n\"C:\\XctAnaDLL\\Common\\Pas\\WinTmr.pas\"\n\"C:\\XctAnaDLL\\Common\\Pas\\WinTools.pas\"\n\"C:\\XctAnaDLL\\Common\\Pas\\WM_AddMessages.pas\"\n\"C:\\XctAnaDLL\\Common\\Pas\\XbJobSel.pas\"\n\"C:\\XctAnaDLL\\Common\\Pas\\XctChecks.pas\"\n\"C:\\XctAnaDLL\\Common\\Pas\\XctDirFrm.pas\"\n\"C:\\XctAnaDLL\\Common\\Pas\\XctLicense.pas\"\n\"C:\\XctAnaDLL\\Common\\Pas\\XctSetStartPosition.pas\"\n\"C:\\XctAnaDLL\\Common\\Pas\\XctVersion.pas\"\n\"C:\\XctAnaDLL\\Common\\Pas\\XGlb.pas\"\n\"C:\\XctAnaDLL\\Common\\Pas\\XGLB_FB.PAS\"\n\"C:\\XctAnaDLL\\Common\\Pas\\XMeasGrp.pas\"\n\"C:\\XctAnaDLL\\Ana\\Pas\\XSETPAR.pas\"\n\"C:\\XctAnaDLL\\Ana\\Pas\\XSETUP.pas\"\n\"C:\\XctAnaDLL\\Ana\\Pas\\XTRACT.pas\""  # Files *.pas
  (unwired) path[] []
  # "FileMapping: only used by XctAnaDLL.dpr"
  # "Look out: some  *.pas files  do  not have a *.dcu file\nwhen included like\n{$I I_Connector_Diff.pas}"
  # "C:\\XctAnaDLL\\Ana\\UNIT\\A_XctDir.dcu"
  # "C:\\XctAnaDLL\\Ana\\FormTranslate.pas"
  n1 = Spreadsheet String To Array(delimiter (Tab)="\n", format string="%s", spreadsheet string=w19, array type (2D Dbl)=string[] []) -> (array=w9:string[])
  n2 = Spreadsheet String To Array(delimiter (Tab)="\n", format string="%s", spreadsheet string=w18, array type (2D Dbl)=string[] []) -> (array=w10:string[])
  n3 = for {
    tunnel: [w32] -> w5 mode=indexing
    tunnel: w9 -> [w28] mode=indexing
    tunnel: [w27] -> _ mode=indexing
    tunnel: [w26] -> w7 mode=indexing
    n4 = Match Pattern(string=w28, regular expression="^[\\t\\n\\r\\s\"]*") -> (after substring=w31:string)  [unwired: 1 in, 3 out]
    n5 = Match Pattern(string=w31, regular expression="[\\t\\n\\r\\s\"]*$") -> (before substring=w26:string)  [unwired: 1 in, 3 out]
    n6 = String To Path(string=w26) -> (path=w27:path)
    n7 = Strip Path(path=w27) -> (name=w33:string)  [unwired: 1 out]
    n8 = call-poly <userlib>:"Strip Path Extension__ogtk.vi"("path"=w33) -> ("root"=w32:string)  [unwired: 1 out]
  }
  "array" <- w7
  n9 = for {
    tunnel: [w40] -> w3 mode=indexing
    tunnel: w10 -> [w36] mode=indexing
    tunnel: [w35] -> w11 mode=indexing
    tunnel: [w34] -> w8 mode=indexing
    n10 = Match Pattern(string=w36, regular expression="^[\\t\\n\\r\\s\"]*") -> (after substring=w39:string)  [unwired: 1 in, 3 out]
    n11 = Match Pattern(string=w39, regular expression="[\\t\\n\\r\\s\"]*$") -> (before substring=w34:string)  [unwired: 1 in, 3 out]
    n12 = String To Path(string=w34) -> (path=w35:path)
    n13 = Strip Path(path=w35) -> (name=w41:string)  [unwired: 1 out]
    n14 = call-poly <userlib>:"Strip Path Extension__ogtk.vi"("path"=w41) -> ("root"=w40:string)  [unwired: 1 out]
  }
  "array 2" <- w8
  n15 = To Upper Case(1:w5) -> (0:w6:string[])
  n16 = To Upper Case(1:w3) -> (0:w4:string[])
  n17 = To Upper Case(1:w2) -> (0:w1:string[])
  n18 = for {
    tunnel: w6 -> [w51]
    tunnel: w4 -> [w46] mode=indexing
    tunnel: w8 -> [w50] mode=indexing
    tunnel: [w50] -> w15 mode=indexing if=w42
    tunnel: [w48] -> w17 mode=indexing if=w42
    tunnel: w11 -> [w48] mode=indexing
    tunnel: w1 -> [w47]
    n19 = Search 1D Array(1D array=w51, element=w46) -> (index of element=w49:i32)  [unwired: 1 in]
    n20 = Search 1D Array(1D array=w47, element=w46) -> (index of element=w45:i32)  [unwired: 1 in]
    n21 = Less Than 0?(x=w49) -> (x < 0?=w43:bool)
    n22 = Less Than 0?(x=w45) -> (x < 0?=w44:bool)
    n23 = Compound Arithmetic op=AND(w43, w44) -> (w42:bool)
  }
  "array 3" <- w15
  n24 = Array To Spreadsheet String(delimiter (Tab)="\n", array=w15, 3:"%s" ("format string")) -> (spreadsheet string=→"spreadsheet string":string)
  n25 = case shown="True" "Delete?" {
    tunnel: w17 -> [_ w52]
    frame False {
    }
    frame True {
      n26 = for {
        tunnel: w52 -> [w53] mode=indexing
        n27 = Delete(path (use dialog)=w53) -> ()  [unwired: 4 in, 3 out]
      }
    }
  }
